vi "Sum of Digits.vi"() -> ()   [LabVIEW 2026]
panel:
  out "Sum Of Digits":dbl
  in  "Input Number(N)":i64
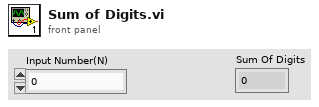
[diagram p1: front panel]
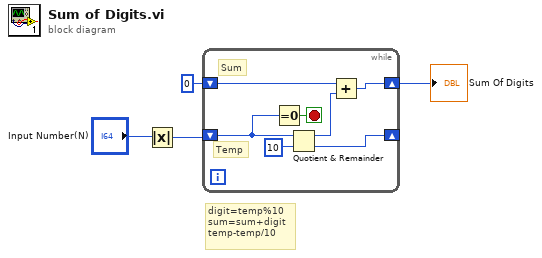
[diagram p0: block diagram]
diagram:
  # "digit=temp%10\nsum=sum+digit\ntemp-temp/10"
  n1 = Absolute Value(x="Input Number(N)") -> (abs(x)=w1:i64)
  n2 = while {
    shift-right: [w10] -> w3
    shift-left: i64 0 -> [w6]
    shift-right: [w9] -> _
    shift-left: w1 -> [w8]
    stop <- w7 stop-if-true
    # "Temp"
    # "Sum"
    n3 = Equal To 0?(x=w8) -> (x = 0?=w7:bool)
    n4 = Quotient & Remainder(x=w8, y=i64 10) -> (x-y*floor(x/y)=w5:i64, floor(x/y)=w9:i64)
    n5 = Add(x=w6, y=w5) -> (x+y=w10:i64)
  }
  "Sum Of Digits" <- w3
